vi "laser_controller_state_machine.vi"() -> ()   [LabVIEW 2025, in "tSNIP.lvlib"]
uses:
  tSNIP.lvlib
panel:
  in  "Laser Mode":enum32{"Calibrate", "Deploy"}(radio)
  in  "error in)":errorcluster
  out "error out":errorcluster
  in  "STOP":bool
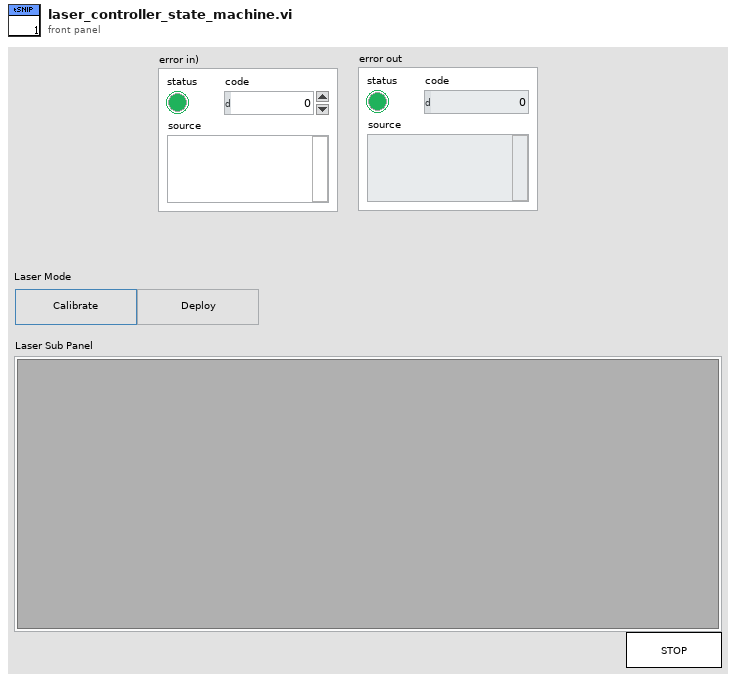
[diagram p1: front panel]
types:
  T1 = enum32{"Bad", "Idle", "Run top level", "Running"}
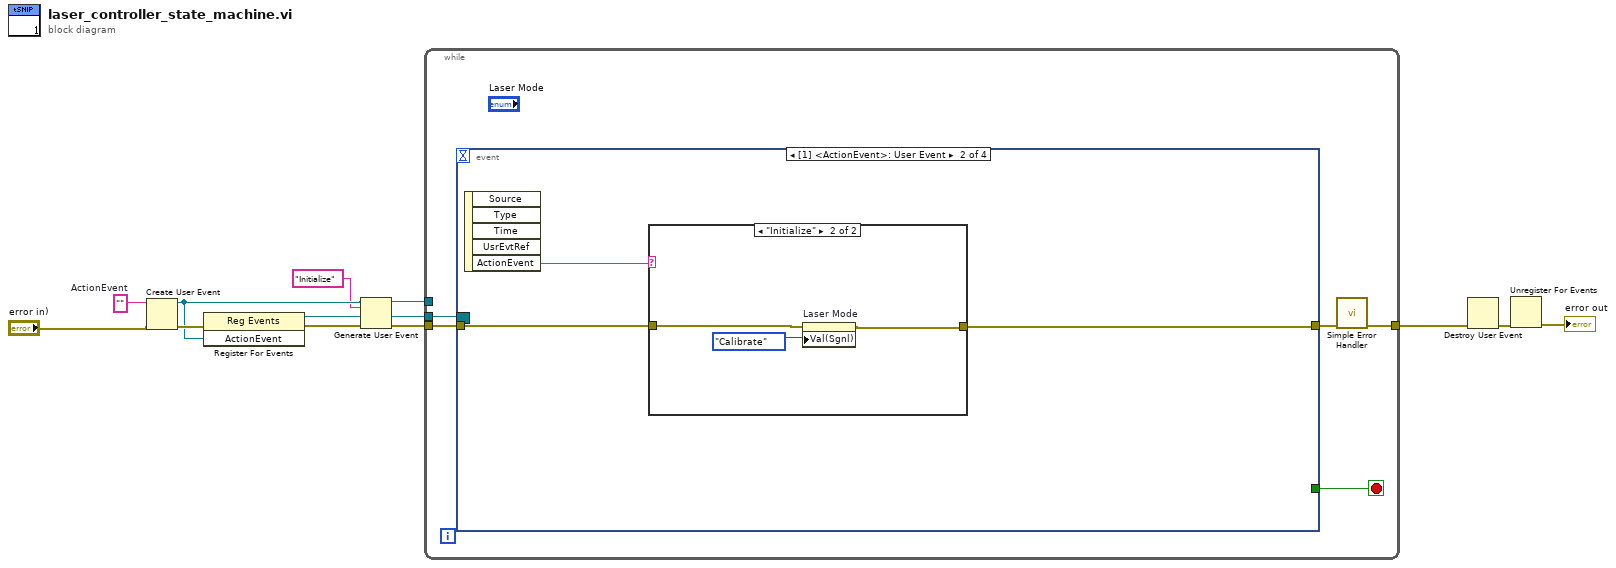
[diagram p0: block diagram]
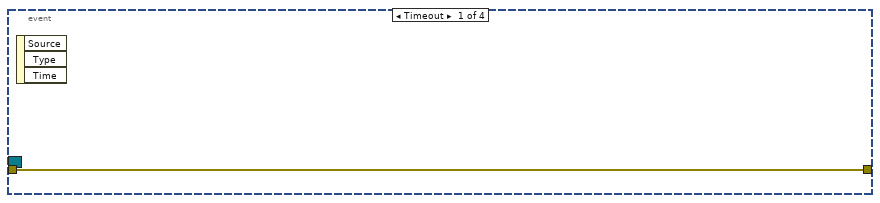
[diagram p2: hidden frame]
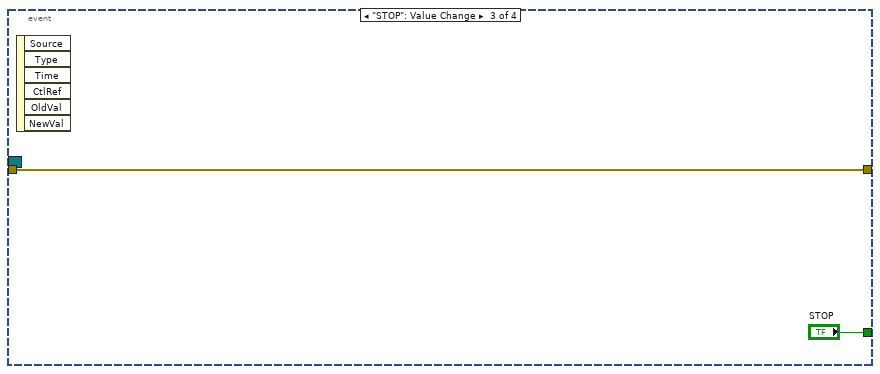
[diagram p4: hidden frame]
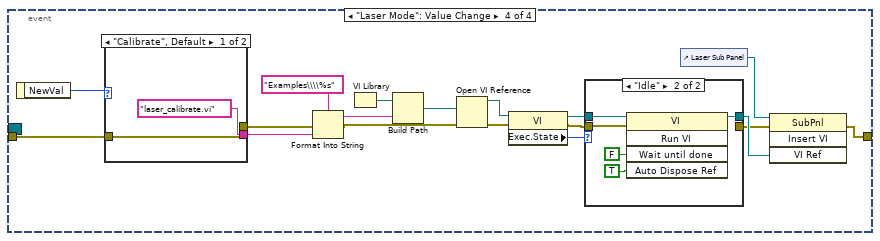
[diagram p5: hidden frame]
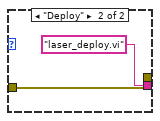
[diagram p7: hidden frame]
diagram:
  w11 = ""  # ActionEvent
  n1 = Create User Event(user event datatype=w11, error in="error in)") -> (user event=w9:refnum<user-event>, error out=w12:errorcluster)
  n2 = register-events(error in=w12, w9) -> (reference out=w8:refnum<event-registration>, error out=w10:errorcluster)  [unwired: 1 in]
  n3 = Generate User Event(user event=w9, event data cluster="Initialize" ("ActionEvent"), error in=w10) -> (user event out=w7:refnum<user-event>, error out=w6:errorcluster)  [unwired: 1 in]
  n4 = while {
    tunnel: w8 -> [w17]
    tunnel: w7 -> [_]
    tunnel: w6 -> [w16]
    tunnel: [w14] -> w3
    stop <- w13 stop-if-true
    n5 = event shown="[1] <ActionEvent>: User Event" {
      selector: w17 -> [_ _ _ _]
      dyn-events: _ -> [_ _ _ _]
      timeout: _ -> [_ _ _ _]
      tunnel: w16 -> [w18 w20 w26 w44]
      tunnel: [w18 w19 w26 w31] -> w15
      tunnel: [_ _ "STOP" _] -> w13
      event Timeout {
        n6 = event-data() -> ()  [unwired: 1 in, 3 out]
      }
      event User Event {
        n7 = event-data() -> ("ActionEvent"=w21:string)  [unwired: 1 in, 4 out]
        n8 = case shown="\"Initialize\"" w21 {
          tunnel: w20 -> [w22 w24]
          tunnel: [w22 w23] -> w19
          frame "False", Default {
            # "TODO: Add error handling"
          }
          frame "Initialize" {
            n9 = property on="Laser Mode" class="RadioBtnsControl (strict)"(error in=w24, "Val(Sgnl)"=enum32{"Calibrate", "Deploy"}."Calibrate" ("Value (Signaling)")) -> (error out=w23:errorcluster)  [unwired: 1 in, 1 out]
          }
        }
      }
      event "STOP": Value Change {
        n10 = event-data() -> ()  [unwired: 1 in, 6 out]
      }
      event "Laser Mode": Value Change {
        n11 = event-data() -> ("NewVal"=w45:enum32{"Calibrate", "Deploy"})  [unwired: 1 in]
        n12 = case shown="\"Calibrate\", Default" w45 {
          tunnel: w44 -> [w53 w56]
          tunnel: [w53 w56] -> w35
          tunnel: ["laser_calibrate.vi" ("ActionEvent") "laser_deploy.vi" ("ActionEvent")] -> w42
          frame "Calibrate", Default {
          }
          frame "Deploy" {
          }
        }
        n13 = Format Into String(format string="Examples\\\\%s", error in=w35, w42) -> (resulting string=w40:string, error out=w38:errorcluster)  [unwired: 1 in]
        n14 = VI Library() -> (path=w41:path)
        n15 = Build Path(base path=w41, name or relative path=w40) -> (appended path=w39:path)
        n16 = Open VI Reference(vi path=w39, error in (no error)=w38) -> (vi reference=w37:refnum<vi>, error out=w36:errorcluster)  [unwired: 4 in]
        n17 = property class="VI"(reference=w37, error in=w36) -> (reference out=w33:refnum<vi>, error out=w32:errorcluster, "Exec.State"=w34:T1)
        n18 = case shown="\"Idle\"" w34 {
          tunnel: w33 -> [w47 w52]
          tunnel: w32 -> [w46 w51]
          tunnel: [w47 w48] -> w29
          tunnel: [w46 _] -> w28
          frame "Bad", Default {
          }
          frame "Idle" {
            n19 = invoke class="VI" method="Run VI"(reference=w52, error in=w51, "Wait until done"=FALSE ("Wait Until Done"), "Auto Dispose Ref"=TRUE ("Auto Dispose Reference")) -> (reference out=w48:refnum<vi>)  [unwired: 1 in, 4 out]
          }
        }
        n20 = control-ref of="Laser Sub Panel"() -> (w30:refnum<vi>)
        n21 = invoke class="SubPnl" method="Insert VI"(reference=w30, error in=w28, "VI Ref"=w29) -> (error out=w31:errorcluster)  [unwired: 1 in, 3 out]
      }
    }
    n22 = call <vilib>:"Simple Error Handler.vi"("error in (no error)"=w15) -> ("error out"=w14:errorcluster)  [unwired: 4 in, 4 out]
  }
  n23 = Destroy User Event(error in=w3) -> (error out=w4:errorcluster)  [unwired: 1 in]
  n24 = Unregister For Events(error in=w4) -> (error out=→"error out":errorcluster)  [unwired: 1 in]
